vi "Test Process Generate Broadcast Event.vi"(8 "error in (no error)":errorcluster, 11 "Process Test In":refnum<class "Process Dev Test.lvclass">) -> (0 "error out":errorcluster, 3 "Process Test Out":refnum<class "Process Dev Test.lvclass">)   [LabVIEW 2020, in "Process Dev Test.lvclass"]
uses:
  Process Dev Test.lvclass
  C:/Program Files (x86)/National Instruments/LabVIEW 2020/vi.lib/Astemes/LUnit/Test Case.lvclass
  source/Framework Test Suite/Mock Process/Mock Process.lvclass
  C:/git/astemes-triarc-framework/source/Framework/Process/Process.lvclass
  source/Framework/Process/Process.lvclass/Process.ctl
  <vilib>/Astemes/LUnit/Test Case.lvclass/Test Case.ctl
  a972513e-0177-4a2b-a6de-788c1d29ea15.vi
  source/Framework/Broadcast Event Dequeuers/Execution timer.vi
  source/Framework/Process/Private/SubVIs/Wait for finish.vi
  source/Framework/Process/Private/SubVIs/Set Lifecycle State.vi
  source/Framework/Process/Protected/Messaging/Send Message.vi
  <vilib>/Astemes/LUnit/Append Pass Result.vi
  <vilib>/Astemes/LUnit/Append Fail Result.vi
  a972513e-0177-4a2b-a6de-788c1d29ea15.vi/9c5d11cd-9439-4240-a1ee-d9baace9c924.vi
  source/Framework/Process/Private/SubVIs/Handle Debug Data.vi
  <vilib>/Astemes/LUnit/Run In UI.vi
  source/Framework/Logging/Log Debug.vi
  <vilib>/AdvancedString/1D String Array to Delimited String.vi
  <vilib>/Utility/High Resolution Relative Seconds.vi
  <vilib>/Utility/error.llb/Clear Errors.vi
  source/Framework/Process/Public/Lifecycle/Get Lifecycle State.vi
  <vilib>/Utility/error.llb/Error Cluster From Error Code.vi
  source/Framework/Process/Public/Read Name.vi
  source/Framework/Broadcast Event Dequeuers/Dequeue Broadcast Message.vi
  source/Framework/Callback/Callback.lvclass
  source/Framework/Process/Process.lvclass
  Process Dev Test.lvclass/Process Dev Test.ctl
  source/Framework/Broadcast Event Dequeuers/Broadcast Event Dequeuers.lvlib
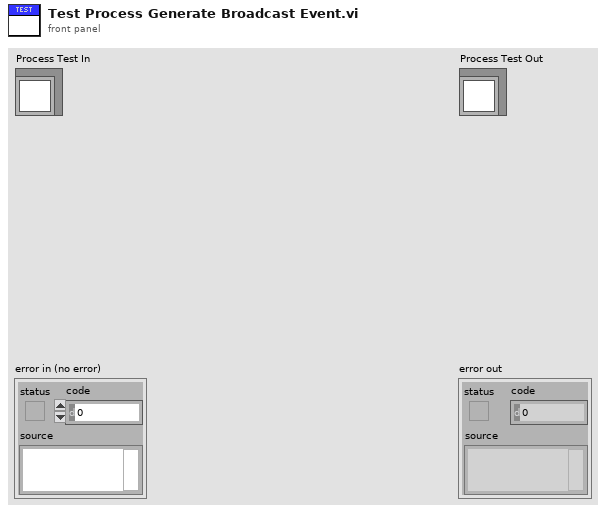
[diagram p1: front panel]
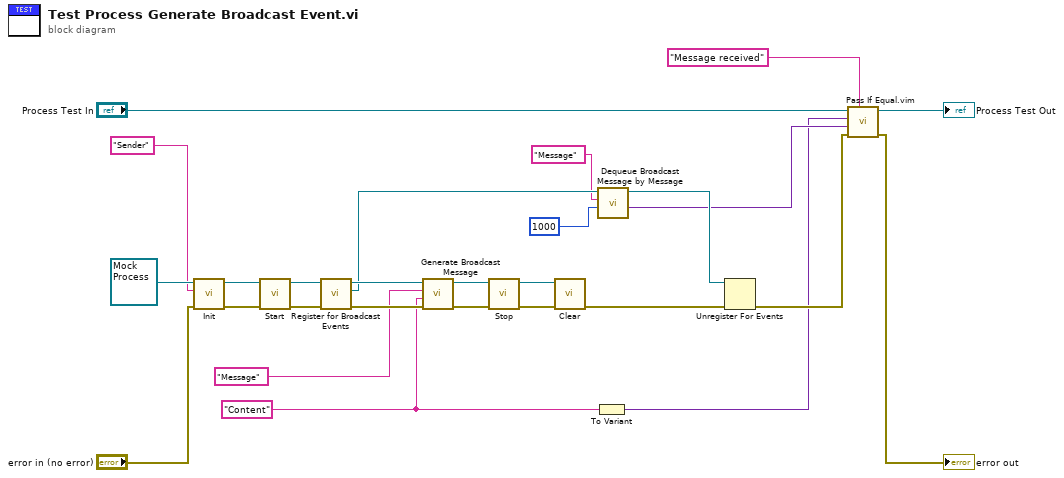
[diagram p0: block diagram]
diagram:
  w12 = "Content" ("Message")
  n1 = call-dynamic "Init.vi"("error in (no error)"="error in (no error)", "Name"="Sender" ("Message"), "Mock Process In"=refnum<class "Mock Process.lvclass"> refnum ("Mock Process.lvclass")) -> ("error out"=w25:errorcluster, "Mock Process Out"=w26:refnum<class "Mock Process.lvclass">)  [unwired: 7 in]
  n2 = call "Start.vi"("error in (no error)"=w25, "Process In"=w26) -> ("error out"=w16:errorcluster, "Process Out"=w18:refnum<class "Mock Process.lvclass">)  [unwired: 7 in, 1 out]
  n3 = call "Register for Broadcast Events.vi"("error in (no error)"=w16, "Process In"=w18) -> ("error out"=w15:errorcluster, "Event Registration Refnum Out"=w14:refnum<event-registration>, "Process Out"=w17:refnum<class "Mock Process.lvclass">)  [unwired: 7 in]
  n4 = call "Generate Broadcast Message.vi"("error in (no error)"=w15, "Message Data"=w12, "Message"="Message", "Mock Process In"=w17) -> ("error out"=w23:errorcluster, "Mock Process Out"=w24:refnum<class "Mock Process.lvclass">)  [unwired: 6 in]
  n5 = call "Stop.vi"("error in (no error)"=w23, "Process In"=w24) -> ("error out"=w22:errorcluster, "Process Out"=w3:refnum<class "Mock Process.lvclass">)  [unwired: 7 in, 1 out]
  n6 = call-dynamic "Clear.vi"("error in (no error)"=w22, "Mock Process In"=w3) -> ("error out"=w21:errorcluster)  [unwired: 9 in]
  n7 = To Variant(anything=w12) -> (Variant=w1:variant)
  n8 = call "Dequeue Broadcast Message by Message.vi"("Timeout (-1)"=1000, "Message"="Message", "Event Registration Refnum"=w14) -> ("Message Data"=w5:variant, "Event Registration Refnum Out"=w13:refnum<event-registration>)  [unwired: 4 in, 3 out]
  n9 = Unregister For Events(event registration refnum=w13, error in=w21) -> (error out=w9:errorcluster)
  n10 = call "Pass If Equal.vim"("Description"="Message received", "error in (no error)"=w9, "Actual"=w5, "Expected"=w1, "LUnit Test Case In"="Process Test In") -> ("error out"=→"error out":errorcluster, "LUnit Test Case Out"=→"Process Test Out":refnum<class "Process Dev Test.lvclass">)  [unwired: 5 in]
